vi "test request status.vi"(8 "error in (no error)":errorcluster) -> (0 "error out":errorcluster, 3 "body":string)   [LabVIEW 2020, in "MCP Server tests.lvlib"]
doc: "A request with an id must be answered with 200 and a JSON-RPC result that carries the same id."
uses:
  MCP Server tests.lvlib
  <vilib>/JDP Science/JSONtext/Next JSON Value.vi
  <vilib>/JDP Science/JSONtext/String Subset.vi
  <vilib>/JDP Science/JSONtext/Parsing/Advance past next JSON Value (inlined COPY).vi
  <vilib>/JDP Science/JSONtext/Parsing/Advance past whitespace.vi
  <vilib>/JDP Science/JSONtext/Parsing/Advance past String.vi
  <vilib>/JDP Science/JSONtext/Parsing/Advance past Number.vi
  <vilib>/JDP Science/JSONtext/Parsing/Advance past Line Ending.vi
  <vilib>/JDP Science/JSONtext/Parsing/Parse Full Path or Item Name.vi
  <vilib>/JDP Science/JSONtext/Parsing/Advance past Array.vi
  <vilib>/JDP Science/JSONtext/Parsing/Advance past Object.vi
  <vilib>/JDP Science/JSONtext/support/Error Cluster From Code.vi
  <vilib>/JDP Science/JSONtext/Offset/Find Item Locations by Path.vi
  <vilib>/addons/_JKI Toolkits/Caraya/classes/Test/Test.lvclass
  <vilib>/JDP Science/JSONtext/JSONtext.lvlib
  <vilib>/addons/_JKI Toolkits/Caraya/classes/Assert/Assert.lvclass
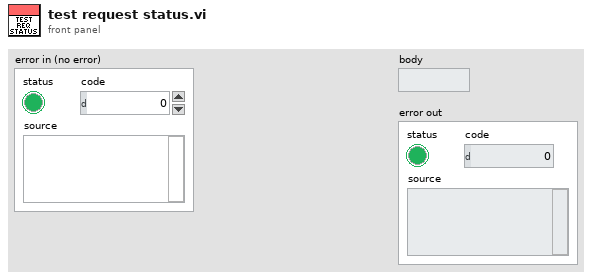
[diagram p1: front panel]
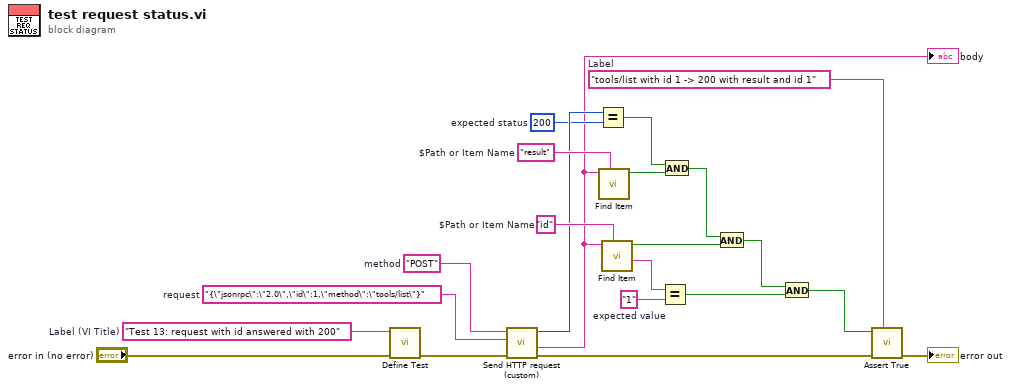
[diagram p0: block diagram]
diagram:
  w3 = "tools/list with id 1 -> 200 with result and id 1"  # Label
  w12 = "1"  # expected value
  w14 = 200  # expected status
  w16 = "id"  # $Path or Item Name
  w17 = "result"  # $Path or Item Name
  w19 = "{\"jsonrpc\":\"2.0\",\"id\":1,\"method\":\"tools/list\"}"  # request
  w20 = "POST"  # method
  w22 = "Test 13: request with id answered with 200"  # Label (VI Title)
  n1 = call <vilib>:"Define Test.vi"("error in (no error)"="error in (no error)", "Label (VI Title)"=w22) -> ("error out"=w18:errorcluster)  [unwired: 8 in, 1 out]
  n2 = call "Send HTTP request (custom).vi"("error in (no error)"=w18, "request"=w19, "method"=w20) -> ("error out"=w4:errorcluster, "response"=w2:string, "status code"=w15:i32)  [unwired: 5 in, 1 out]
  "body" <- w2
  n3 = Equal?(x=w15, y=w14) -> (x = y?=w11:bool)
  n4 = call <vilib>:"Find Item.vi"("$Path or Item Name"=w17, "JSON"=w2) -> ("Found"=w10:bool)  [unwired: 6 in, 3 out]
  n5 = call <vilib>:"Find Item.vi"("$Path or Item Name"=w16, "JSON"=w2) -> ("<JSON>"=w13:string, "Found"=w8:bool)  [unwired: 6 in, 2 out]
  n6 = Equal?(x=w13, y=w12) -> (x = y?=w6:bool)
  n7 = And(x=w11, y=w10) -> (x .and. y?=w9:bool)
  n8 = And(x=w9, y=w8) -> (x .and. y?=w7:bool)
  n9 = And(x=w7, y=w6) -> (x .and. y?=w5:bool)
  n10 = call <vilib>:"Assert True.vi"("Label"=w3, "error in (no error)"=w4, "True?"=w5) -> ("error out"=→"error out":errorcluster)  [unwired: 7 in, 1 out]
